vi "Enregis fichier logbook.vi"(2 "entrée d'erreur":errorcluster, 3 "Chaîne":string) -> (0 "sortie d'erreur":errorcluster)   [LabVIEW 2022 SP3]
uses:
  Variables globales/Variable glob generale.vi
panel:
  # "enregistrer dans fichier logbook"
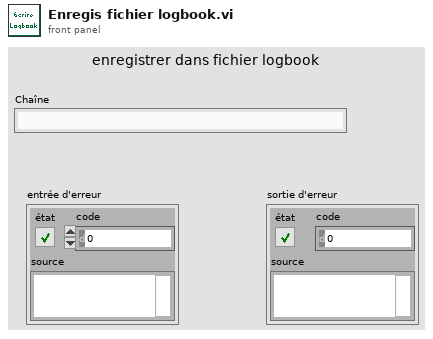
[diagram p1: front panel]
types:
  T1 = enum16{"open", "replace", "create", "open or create", "replace or create", "replace or create with confirmation"}
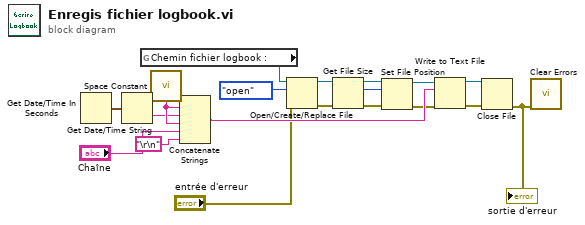
[diagram p0: block diagram]
diagram:
  n1 = Get Date/Time In Seconds() -> (seconds since 1Jan1904=w14:timestamp)
  n2 = Get Date/Time String(seconds (now)=w14) -> (date string=w15:string, time string=w16:string)  [unwired: 2 in]
  n3 = global read "Variable glob generale.vi" "Chemin fichier logbook :"() -> (w2:path)
  n4 = call <vilib>:"Space Constant.vi"() -> ("String"=w17:string)
  n5 = Concatenate Strings(w15, w17, w16, w17, "Chaîne", "\r\n") -> (w20:string)
  n6 = Open/Create/Replace File(file path (use dialog)=w2, error in="entrée d'erreur", operation (0:open)=T1."open" ("opération (0 : open)")) -> (refnum out=w7:refnum<file>, error out=w8:errorcluster)  [unwired: 4 out]
  n7 = Get File Size(file=w7, error in=w8) -> (refnum out=w11:refnum<file>, size (in bytes)=w10:i64, 0:w9:errorcluster)
  n8 = Set File Position(offset (in bytes) (0)=w10, refnum=w11, error in=w9) -> (refnum out=w12:refnum<file>, error out=w13:errorcluster)  [unwired: 1 in]
  n9 = Write to Text File(file (use dialog)=w12, text=w20, error in=w13) -> (refnum out=w4:refnum<file>, error out=w5:errorcluster)  [unwired: 1 in, 1 out]
  n10 = Close File(refnum=w4, error in=w5) -> (error out=w3:errorcluster)  [unwired: 1 out]
  "sortie d'erreur" <- w3
  n11 = call <vilib>:"Clear Errors.vi"("error in (no error)"=w3) -> ()  [unwired: 5 in, 2 out]
